vi "current_pulse_train_timed.vi"(0 "Current Train Ref":refnum<vi>, 1 "Laser Active Ref":refnum<vi>, 5 "Elapsed Time Ref":refnum<vi>, 7 "Instantaneous Current Ref":refnum<vi>, 9 "Current Waveform Ref":refnum<vi>, 11 "error in":errorcluster, 12 "Exit Ref":refnum<vi>) -> (15 "error out":errorcluster)   [LabVIEW 2025, in "tSNIP.lvlib"]
uses:
  tSNIP.lvlib
panel:
  out "Instantaneous Current":cluster{"Value":dbl, "Units":dbl}={"Value"=0.0, "Units"=0.001} {"Units" items=["mA"=0.001, "A"=1.0]}
  out "Number of Cycles":u64
  out "Elapsed time":dbl format="%<%M:%S>t"
  out "Current Waveform":waveform(dbl)(graph)
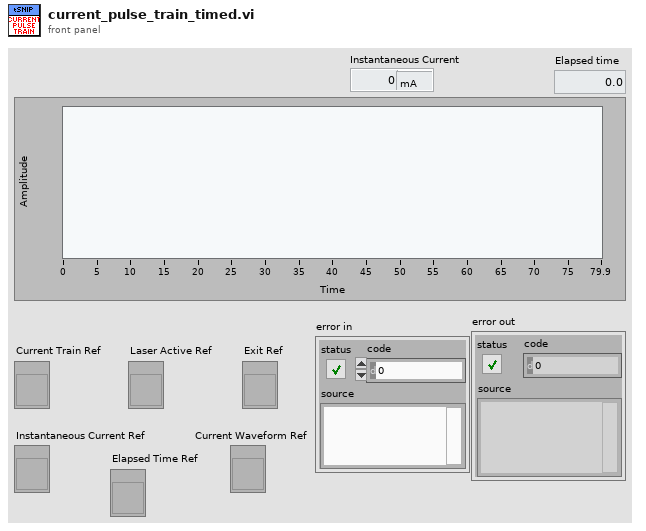
[diagram p1: front panel]
types:
  T1 = cluster{"Duty Cycle":cluster{"ON":cluster{"Units":u16, "Value":dbl}, "OFF":cluster{"Units":u16, "Value":dbl}}, "Number of Cycles":u64, "Current Step":cluster{"Value":dbl, "Units":dbl}, "Start Current":cluster{"Value":dbl, "Units":dbl}}
  T2 = cluster{"ON":cluster{"Units":u16, "Value":dbl}, "OFF":cluster{"Units":u16, "Value":dbl}}
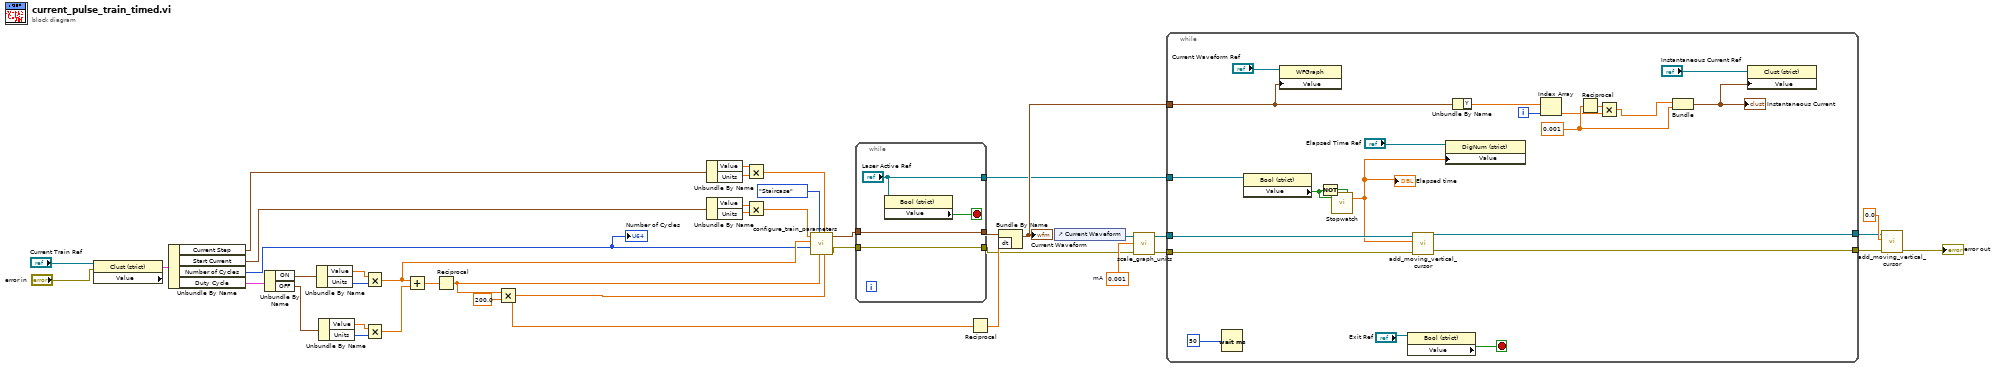
[diagram p0: block diagram]
diagram:
  w41 = 0.001  # mA
  n1 = property class="Clust (strict)"(reference="Current Train Ref", error in="error in") -> ("Value"=w23:T1)  [unwired: 2 out]
  n2 = Unbundle By Name(w23) -> ("Current Step"=w21:cluster{"Value":dbl, "Units":dbl}, "Start Current"=w20:cluster{"Value":dbl, "Units":dbl}, "Number of Cycles"=w15:u64, "Duty Cycle"=w34:T2)
  "Number of Cycles" <- w15
  n3 = Unbundle By Name(w34) -> ("ON"=w31:cluster{"Units":u16, "Value":dbl}, "OFF"=w30:cluster{"Units":u16, "Value":dbl})
  n4 = Unbundle By Name(w31) -> ("Value"=w29:dbl, "Units"=w28:u16)
  n5 = Unbundle By Name(w30) -> ("Value"=w27:dbl, "Units"=w26:u16)
  n6 = Multiply(x=w29, y=w28) -> (x*y=w39:dbl)
  n7 = Multiply(x=w27, y=w26) -> (x*y=w40:dbl)
  n8 = Add(x=w39, y=w40) -> (x+y=w11:dbl)
  n9 = Reciprocal(x=w11) -> (1/x=w37:dbl)
  n10 = Multiply(x=w37, y=200.0) -> (x*y=w36:dbl)
  n11 = Unbundle By Name(w21) -> ("Value"=w19:dbl, "Units"=w18:dbl)
  n12 = Unbundle By Name(w20) -> ("Value"=w17:dbl, "Units"=w16:dbl)
  n13 = Multiply(x=w19, y=w18) -> (x*y=w33:dbl)
  n14 = Multiply(x=w17, y=w16) -> (x*y=w32:dbl)
  n15 = call "configure_train_parameters.vi"("Fs"=w36, "Amplitude Step"=w33, "Frequency"=w37, "Current Type"=enum32{"Constant", "Staircase"}."Staircase", "NumCycles"=w15, "Pulse width"=w39, "Amplitude"=w32) -> ("error out"=w10:errorcluster, "Output train"=w8:waveform(dbl))  [unwired: 3 in]
  n16 = while {
    tunnel: w10 -> [w45]
    tunnel: [w45] -> w9
    tunnel: [w44] -> w7
    tunnel: w8 -> [w44]
    tunnel: ["Laser Active Ref"] -> w6
    stop <- w42 stop-if-true
    n17 = property class="Bool (strict)"(reference="Laser Active Ref") -> ("Value"=w42:bool)  [unwired: 1 in, 2 out]
  }
  n18 = Reciprocal(x=w36) -> (1/x=w35:dbl)
  n19 = Bundle By Name(cluster=w7, "dt"=w35) -> (w14:waveform(dbl))
  "Current Waveform" <- w14
  n20 = control-ref of="Current Waveform"() -> (w13:refnum<vi>)
  n21 = call "scale_graph_units.vi"("error in"=w9, "y-units"=w41, "reference in"=w13) -> ("error out"=w3:errorcluster, "reference out"=w12:refnum<vi>)  [unwired: 6 in]
  n22 = while {
    tunnel: w14 -> [w52]
    tunnel: w12 -> [w59]
    tunnel: w6 -> [w50]
    tunnel: [w48] -> w4
    tunnel: w3 -> [w47]
    tunnel: [w46] -> w1
    i -> [w65]
    stop <- w66 stop-if-true
    w62 = 0.001 ("Units")
    n23 = Wait (ms)(milliseconds to wait=u32 50) -> ()  [unwired: 1 out]
    n24 = property class="Bool (strict)"(reference=w50) -> ("Value"=w54:bool)  [unwired: 1 in, 2 out]
    n25 = property class="WFGraph"(reference="Current Waveform Ref", "Value"=w52) -> ()  [unwired: 1 in, 2 out]
    n26 = Not(x=w54) -> (.not. x?=w55:bool)
    n27 = call "Stopwatch.vi"("Start"=w54, "Reset"=w55) -> ("time"=w56:dbl)  [unwired: 17 in]
    "Elapsed time" <- w56
    n28 = property class="Bool (strict)"(reference="Exit Ref") -> ("Value"=w66:bool)  [unwired: 1 in, 2 out]
    n29 = call "add_moving_vertical_cursor.vi"("error in"=w47, "Cursor Position"=w56, "reference in"=w59) -> ("error out"=w48:errorcluster, "reference out"=w46:refnum<vi>)  [unwired: 7 in]
    n30 = property class="DigNum (strict)"(reference="Elapsed Time Ref", "Value"=w56) -> ()  [unwired: 1 in, 2 out]
    n31 = Unbundle By Name(w52) -> ("Y"=w53:dbl[])
    n32 = Index Array(array=w53, index=w65) -> (element=w51:dbl)
    n33 = Reciprocal(x=w62) -> (1/x=w64:dbl)
    n34 = Multiply(x=w64, y=w51) -> (x*y=w63:dbl)
    n35 = Bundle(w63, "Units"=w62) -> (w57:cluster{dbl, "Units":dbl})  [unwired: 1 in]
    "Instantaneous Current" <- w57
    n36 = property class="Clust (strict)"(reference="Instantaneous Current Ref", "Value"=w57) -> ()  [unwired: 1 in, 2 out]
  }
  n37 = call "add_moving_vertical_cursor.vi"("error in"=w4, "Cursor Position"=0.0, "reference in"=w1) -> ("error out"=→"error out":errorcluster)  [unwired: 7 in, 1 out]
